vi "Create Raw Writer.vi"(6 "Descriptor":string, 8 "error in (no error)":errorcluster, 9 "Data":u8[](array[numeric]) format="%.0x", 10 "Topic Name":T1, 11 "BlackBoard Reference":T2 {"refnum" format="%.0x"}) -> (0 "error out":errorcluster, 2 "Type Name":string, 3 "Raw Writer Reference":T3 {"refnum" format="%.0x"})   [LabVIEW 2021, in "Iceoryx.lvlib"]
doc: "Blackboard reference: refnum provided from the Blackboard Open\nTopic Name: Topic name is required, Type override is required\nData: The data for the topic. The fixed size is deteremined by the size of the provided array.\n\nRaw writer does not support variable size data and must always write the full array. It is 2x as effecient as it removes a mem copy."
uses:
  Iceoryx.lvlib
  Refnum/Typedef/BB Raw Writer Refnum.ctl
  Refnum/Typedef/BB Refnum.ctl
  typedef/Topic Full Names.ctl
  typedef/Errors.ctl
  SubVIs/Add Error Core.vi
  SubVIs/Convert Error Core.vi
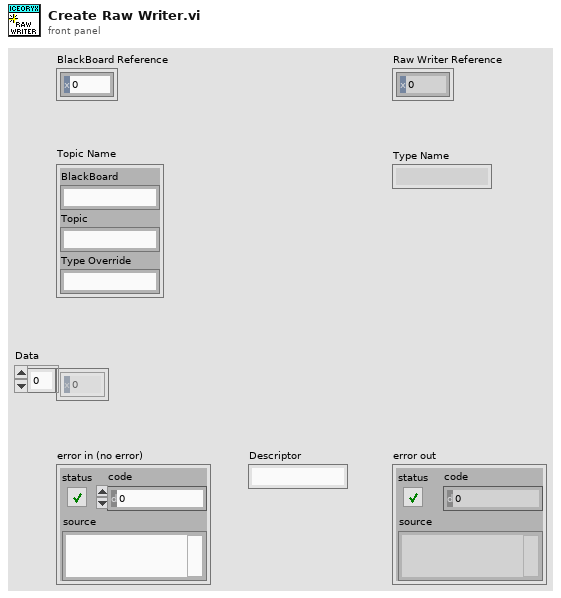
[diagram p1: front panel]
types:
  T1 = typedef "Iceoryx.lvlib/Topic Full Names.ctl" = cluster{"BlackBoard":string, "Topic":string, "Type Override":string}
  T2 = typedef "Iceoryx.lvlib/BB Refnum.ctl" = cluster{"refnum":u64, "BB":enum8{"bb"}}
  T3 = typedef "Iceoryx.lvlib/BB Raw Writer Refnum.ctl" = cluster{"refnum":u64, "BB Raw Writer":enum8{"bb_raw_writer"}}
  T4 = typedef "Iceoryx.lvlib/Errors.ctl" = enum16{"Unsupported Type", "Empty Name", "Cluster Name"}
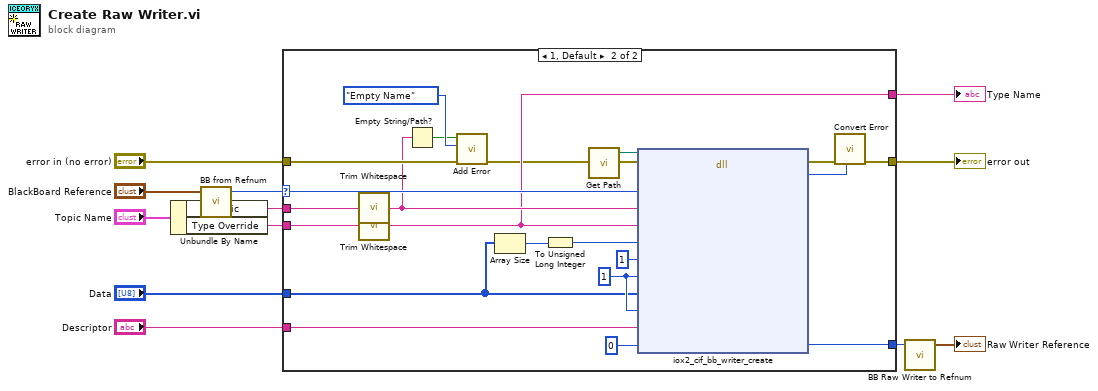
[diagram p0: block diagram]
diagram:
  n1 = Unbundle By Name("Topic Name") -> ("Topic"=w5:string, "Type Override"=w6:string)
  n2 = call "BB from Refnum.vi"("BB Refnum"="BlackBoard Reference") -> ("BB U64"=w3:u64)  [unwired: 4 in]
  n3 = case shown="1, Default" w3 {
    selector: w3 -> [_ w28]
    tunnel: "error in (no error)" -> [w13 w26]
    tunnel: [_ w34] -> w11
    tunnel: [w13 w29] -> w10
    tunnel: "Data" -> [_ w16]
    tunnel: w5 -> [_ w23]
    tunnel: w6 -> [_ w22]
    tunnel: [_ w19] -> w7
    tunnel: "Descriptor" -> [_ w18]
    frame 0 {
    }
    frame 1, Default {
      w21 = u32 1 ("initial_count")
      n4 = call <vilib>:"Trim Whitespace.vi"("string"=w23) -> ("trimmed string"=w24:string)  [unwired: 1 in]
      n5 = call <vilib>:"Trim Whitespace.vi"("string"=w22) -> ("trimmed string"=w19:string)  [unwired: 1 in]
      n6 = Empty String/Path?(string/path=w24) -> (empty?=w25:bool)
      n7 = call "Add Error.vi"("error in (no error)"=w26, "Error"=Errors."Empty Name", "Insert Error"=w25) -> ("error out"=w17:errorcluster)  [unwired: 8 in]
      n8 = Array Size(array=w16) -> (size(s)=w15:i32)
      n9 = To Unsigned Long Integer(number=w15) -> (unsigned 32bit integer=w14:u32)
      n10 = call "Get Path.vi"() -> ("libiox2_cif path"=w32:path)  [unwired: 4 in]
      n11 = dll-call lib="D:/dev/iceoryx2_lvwrapper/dist/iox2_cif.dll" fn="iox2_cif_bb_writer_create"(path in=w32, error in=w17, "bb"=w28, "topic"=w24, "type_name"=w19, "elem_size"=w14, "elem_align"=u32 1, "max_count"=w21, "initial"=w16, "initial_count"=w21, "descriptor"=w18, "writer"=u64 0) -> (error out=w31:errorcluster, "return type"=w30:i32, "writer"=w34:u64)  [unwired: 10 in, 1 out]
      n12 = call "Convert Error.vi"("return type"=w30, "error in (no error)"=w31) -> ("error out"=w29:errorcluster)  [unwired: 9 in]
    }
  }
  "error out" <- w10
  "Type Name" <- w7
  n13 = call "BB Raw Writer to Refnum.vi"("BB Raw Writer U64"=w11) -> ("BB Raw Writer Refnum"=→"Raw Writer Reference":T3)  [unwired: 4 in]
